vi "RDV-addDataToSmithPlot.vi"(8 "error in (no error)":errorcluster, 11 "RDV-Reflection_Data_viewer in":refnum<class "RDV-Reflection_Data_viewer.lvclass">) -> (0 "error out":errorcluster, 3 "RDV-Reflection_Data_viewer out":refnum<class "RDV-Reflection_Data_viewer.lvclass">)   [LabVIEW 2020, in "RDV-Reflection_Data_viewer.lvclass"]
doc: "Writes the reflection data of the viewer's map to its Smith plot."
uses:
  RDV-Reflection_Data_viewer.lvclass
  RDV-Reflection_Data_viewer.lvclass/RDV-Reflection_Data_viewer.ctl
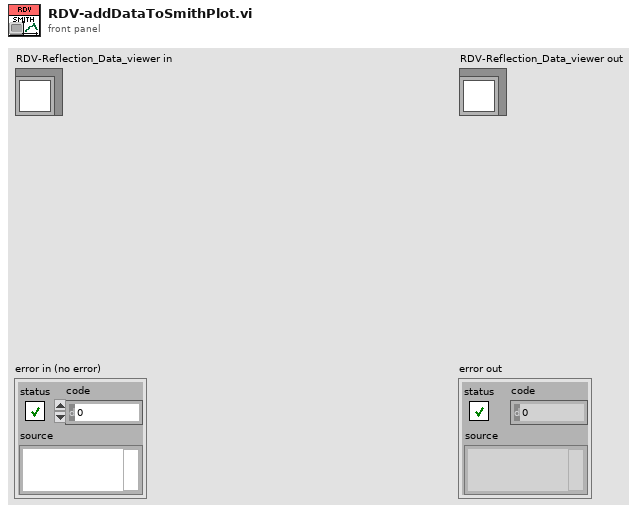
[diagram p1: front panel]
types:
  T1 = cluster{"left":i16, "top":i16, "right":i16, "bottom":i16}
  T2 = cluster{"x minimum":dbl, "x maximum":dbl, "y minimum":dbl, "y maximum":dbl}
  T3 = cluster{"Frequency":dbl[], "Reflection'":dbl[]}[]
  T4 = cluster{"normalized smith points {r,x}":cluster{"r":dbl, "x":dbl}[]}
  T5 = cluster{"ref":u16, "Plot.Plot Color":u32, "Plot.Plot Color":u32}
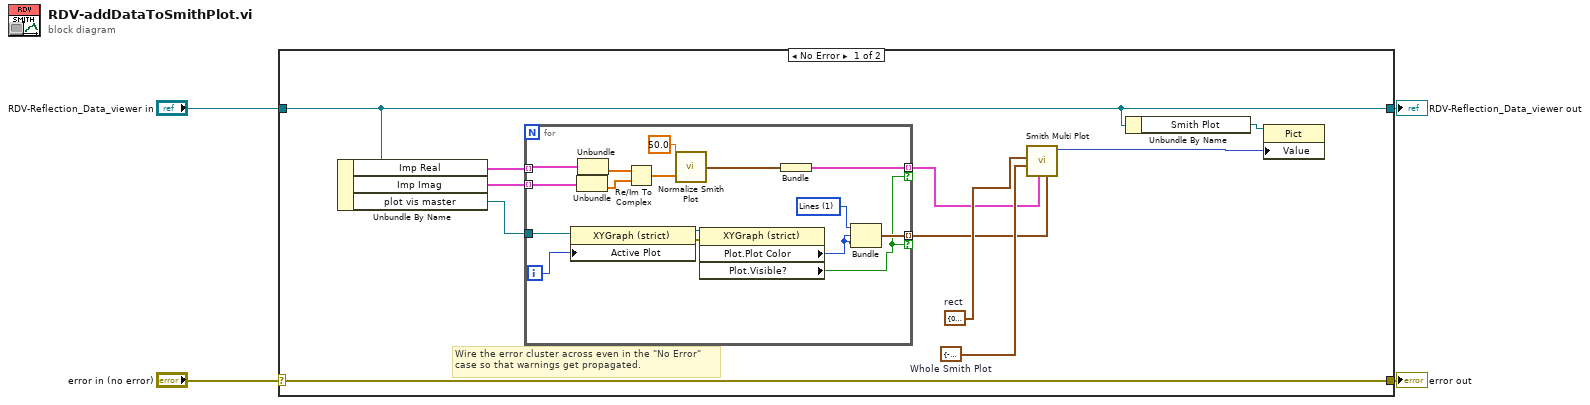
[diagram p0: block diagram]
diagram:
  n1 = case shown="No Error" "error in (no error)" {
    selector: "error in (no error)" -> [w15 w33]
    tunnel: [w15 w33] -> w3
    tunnel: [w7 w32] -> w1
    tunnel: "RDV-Reflection_Data_viewer in" -> [w7 w32]
    frame No Error {
      w10 = T1 {"left"=0, "top"=0, "right"=500, "bottom"=500}  # rect
      w11 = T2 {"x minimum"=-1.0, "x maximum"=1.0, "y minimum"=-1.0, "y maximum"=1.0}  # Whole Smith Plot
      # "Wire the error cluster across even in the \"No Error\"\ncase so that warnings get propagated."
      n2 = Unbundle By Name(w7) -> ("Imp Real"=w14:T3, "Imp Imag"=w13:T3, "plot vis master"=w12:refnum<vi>)
      n3 = for {
        tunnel: w14 -> [w31] mode=indexing
        tunnel: w13 -> [w30] mode=indexing
        tunnel: w12 -> [w23]
        tunnel: [w19] -> w8 mode=indexing if=w16
        tunnel: [w18] -> w9 mode=indexing if=w16
        i -> [w22]
        w21 = u16 1 items=["Points", "Lines", "Points & Lines"] ("ref")
        n4 = property class="XYGraph (strict)"(reference=w23, "Active Plot"=w22) -> (reference out=w25:refnum<vi>, error out=w24:errorcluster)  [unwired: 1 in]
        n5 = Unbundle(w30) -> ("Reflection'"=w27:dbl[])  [unwired: 1 out]
        n6 = Unbundle(w31) -> ("Reflection'"=w28:dbl[])  [unwired: 1 out]
        n7 = Re/Im To Complex(1:w27, 2:w28) -> (0:w26:cdb[])
        n8 = call <vilib>:"Normalize Smith Plot.vi"("points complex"=w26, "Zo (50.0)"=50.0) -> ("normalized smith points {r,x}"=w17:cluster{"r":dbl, "x":dbl}[])  [unwired: 1 in]
        n9 = property class="XYGraph (strict)"(reference=w25, error in=w24) -> ("Plot.Plot Color"=w20:u32, "Plot.Visible?"=w16:bool)  [unwired: 2 out]
        n10 = Bundle("normalized smith points {r,x}"=w17) -> (w18:T4)  [unwired: 1 in]
        n11 = Bundle("ref"=w21, "Plot.Plot Color"=w20, "Plot.Plot Color"=w20) -> (w19:T5)  [unwired: 1 in]
      }
      n12 = call <vilib>:"Smith Multi Plot.vi"("smith plot cosmetics"=w8, "smith multi plot"=w9, "smith plot section"=w11, "rect"=w10) -> ("new picture"=w5:picture)  [unwired: 7 in]
      n13 = Unbundle By Name(w7) -> ("Smith Plot"=w6:refnum<vi>)
      n14 = property class="Pict"(reference=w6, "Value"=w5) -> ()  [unwired: 1 in, 2 out]
    }
    frame Error {
    }
  }
  "error out" <- w3
  "RDV-Reflection_Data_viewer out" <- w1
